vi "Multiple_Ramps_Trimming_Coil.vi"(0 "Trimming_Coil_Ramp_Error":dbl, 1 "Trimming_Coil_Ramp_Inc/Dec":dbl) -> ()   [LabVIEW 2025]
uses:
  Trimming_Coil_Command.vi
  Trimming_Coil_Ramps.vi
panel:
  out "TC1_Set_Point":dbl
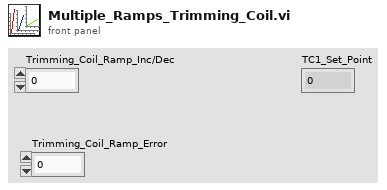
[diagram p1: front panel]
types:
  T1 = cluster{"TC1_Set_Point":dbl, "TC2_Set_Point":dbl, "TC3_Set_Point":dbl, "TC4_Set_Point":dbl, "TC5_Set_Point":dbl, "TC6_Set_Point":dbl, "TC7_Set_Point":dbl, "TC8_Set_Point":dbl, "TC9_Set_Point":dbl, "TC10_Set_Point":dbl, "TC11_Set_Point":dbl, "TC12_Set_Point":dbl}
  T2 = cluster{"TC1_Ramp":dbl, "TC2_Ramp":dbl, "TC3_Ramp":dbl, "TC4_Ramp":dbl, "TC5_Ramp":dbl, "TC6_Ramp":dbl, "TC7_Ramp":dbl, "TC8_Ramp":dbl, "TC9_Ramp":dbl, "TC10_Ramp":dbl, "TC11_Ramp":dbl, "TC12_Ramp":dbl}
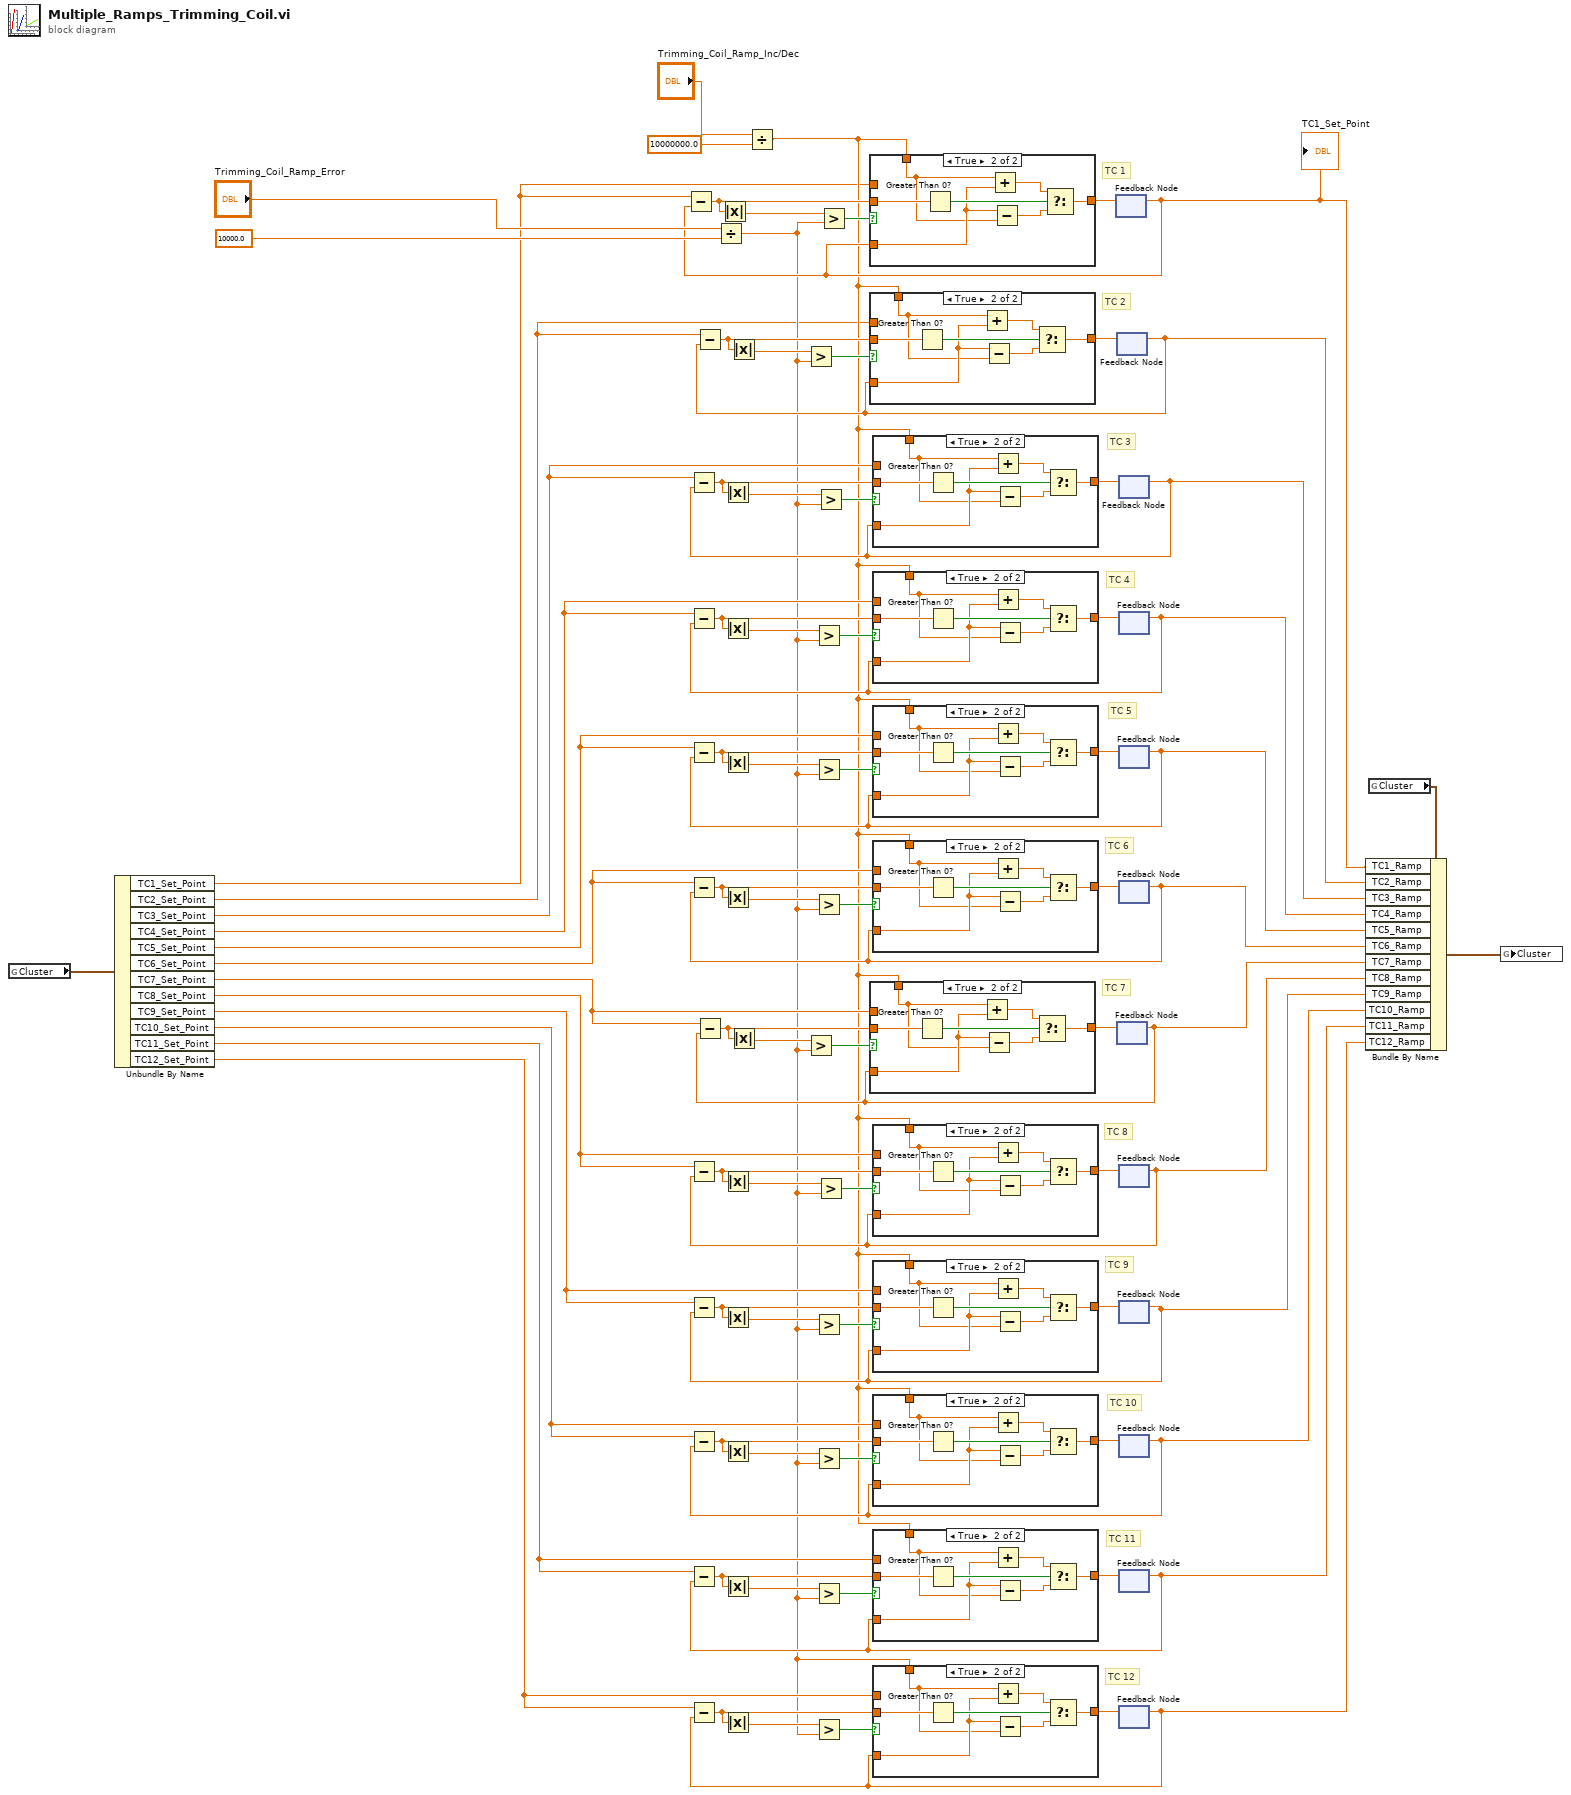
[diagram p0: block diagram]
diagram:
  # "TC 12"
  # "TC 11"
  # "TC 10"
  # "TC 9"
  # "TC 8"
  # "TC 7"
  # "TC 6"
  # "TC 5"
  # "TC 4"
  # "TC 3"
  # "TC 2"
  # "TC 1"
  n1 = global read "Trimming_Coil_Command.vi" "Cluster"() -> (w75:T1)
  n2 = Unbundle By Name(w75) -> ("TC1_Set_Point"=w1:dbl, "TC2_Set_Point"=w2:dbl, "TC3_Set_Point"=w63:dbl, "TC4_Set_Point"=w58:dbl, "TC5_Set_Point"=w49:dbl, "TC6_Set_Point"=w48:dbl, "TC7_Set_Point"=w24:dbl, "TC8_Set_Point"=w23:dbl, "TC9_Set_Point"=w22:dbl, "TC10_Set_Point"=w21:dbl, "TC11_Set_Point"=w20:dbl, "TC12_Set_Point"=w15:dbl)
  n3 = Divide(x="Trimming_Coil_Ramp_Error", y=10000.0) -> (x/y=w3:dbl)
  n4 = Divide(x="Trimming_Coil_Ramp_Inc/Dec", y=10000000.0) -> (x/y=w4:dbl)
  n5 = feedback #1() -> (w5:dbl)  [unwired: 1 in]
  "TC1_Set_Point" <- w5
  n6 = Subtract(x=w1, y=w5) -> (x-y=w80:dbl)
  n7 = Absolute Value(x=w80) -> (abs(x)=w81:dbl)
  n8 = Greater?(x=w81, y=w3) -> (0:w79:bool)
  n9 = case shown="True" w79 {
    tunnel: w80 -> [_ w89]
    tunnel: w5 -> [_ w87]
    tunnel: [w82 w84] -> w78
    tunnel: w1 -> [w82 _]
    tunnel: w4 -> [_ w83]
    frame False {
    }
    frame True {
      n10 = Greater Than 0?(x=w89) -> (x > 0?=w88:bool)
      n11 = Add(x=w83, y=w87) -> (x+y=w85:dbl)
      n12 = Subtract(x=w87, y=w83) -> (x-y=w86:dbl)
      n13 = Select(t=w85, s=w88, f=w86) -> (s? t:f=w84:dbl)
    }
  }
  n14 = feedback-in #1(w78) -> ()
  n15 = feedback #2() -> (w6:dbl)  [unwired: 1 in]
  n16 = Subtract(x=w2, y=w6) -> (x-y=w70:dbl)
  n17 = Absolute Value(x=w70) -> (abs(x)=w71:dbl)
  n18 = Greater?(x=w71, y=w3) -> (0:w69:bool)
  n19 = case shown="True" w69 {
    tunnel: w70 -> [_ w97]
    tunnel: w6 -> [_ w95]
    tunnel: [w90 w92] -> w68
    tunnel: w2 -> [w90 _]
    tunnel: w4 -> [_ w91]
    frame False {
    }
    frame True {
      n20 = Greater Than 0?(x=w97) -> (x > 0?=w96:bool)
      n21 = Add(x=w91, y=w95) -> (x+y=w93:dbl)
      n22 = Subtract(x=w95, y=w91) -> (x-y=w94:dbl)
      n23 = Select(t=w93, s=w96, f=w94) -> (s? t:f=w92:dbl)
    }
  }
  n24 = feedback-in #2(w68) -> ()
  n25 = feedback #3() -> (w14:dbl)  [unwired: 1 in]
  n26 = Subtract(x=w24, y=w14) -> (x-y=w43:dbl)
  n27 = Absolute Value(x=w43) -> (abs(x)=w44:dbl)
  n28 = Greater?(x=w44, y=w3) -> (0:w42:bool)
  n29 = case shown="True" w42 {
    tunnel: w43 -> [_ w105]
    tunnel: w14 -> [_ w103]
    tunnel: [w98 w100] -> w41
    tunnel: w24 -> [w98 _]
    tunnel: w4 -> [_ w99]
    frame False {
    }
    frame True {
      n30 = Greater Than 0?(x=w105) -> (x > 0?=w104:bool)
      n31 = Add(x=w99, y=w103) -> (x+y=w101:dbl)
      n32 = Subtract(x=w103, y=w99) -> (x-y=w102:dbl)
      n33 = Select(t=w101, s=w104, f=w102) -> (s? t:f=w100:dbl)
    }
  }
  n34 = feedback-in #3(w41) -> ()
  n35 = feedback #4() -> (w7:dbl)  [unwired: 1 in]
  n36 = Subtract(x=w63, y=w7) -> (x-y=w66:dbl)
  n37 = Absolute Value(x=w66) -> (abs(x)=w67:dbl)
  n38 = Greater?(x=w67, y=w3) -> (0:w65:bool)
  n39 = case shown="True" w65 {
    tunnel: w66 -> [_ w113]
    tunnel: w7 -> [_ w111]
    tunnel: [w106 w108] -> w64
    tunnel: w63 -> [w106 _]
    tunnel: w4 -> [_ w107]
    frame False {
    }
    frame True {
      n40 = Greater Than 0?(x=w113) -> (x > 0?=w112:bool)
      n41 = Add(x=w107, y=w111) -> (x+y=w109:dbl)
      n42 = Subtract(x=w111, y=w107) -> (x-y=w110:dbl)
      n43 = Select(t=w109, s=w112, f=w110) -> (s? t:f=w108:dbl)
    }
  }
  n44 = feedback-in #4(w64) -> ()
  n45 = feedback #5() -> (w47:dbl)  [unwired: 1 in]
  n46 = Subtract(x=w58, y=w47) -> (x-y=w61:dbl)
  n47 = Absolute Value(x=w61) -> (abs(x)=w62:dbl)
  n48 = Greater?(x=w62, y=w3) -> (0:w60:bool)
  n49 = case shown="True" w60 {
    tunnel: w61 -> [_ w121]
    tunnel: w47 -> [_ w119]
    tunnel: [w114 w116] -> w59
    tunnel: w58 -> [w114 _]
    tunnel: w4 -> [_ w115]
    frame False {
    }
    frame True {
      n50 = Greater Than 0?(x=w121) -> (x > 0?=w120:bool)
      n51 = Add(x=w115, y=w119) -> (x+y=w117:dbl)
      n52 = Subtract(x=w119, y=w115) -> (x-y=w118:dbl)
      n53 = Select(t=w117, s=w120, f=w118) -> (s? t:f=w116:dbl)
    }
  }
  n54 = feedback-in #5(w59) -> ()
  n55 = feedback #6() -> (w46:dbl)  [unwired: 1 in]
  n56 = Subtract(x=w49, y=w46) -> (x-y=w56:dbl)
  n57 = Absolute Value(x=w56) -> (abs(x)=w57:dbl)
  n58 = Greater?(x=w57, y=w3) -> (0:w55:bool)
  n59 = case shown="True" w55 {
    tunnel: w56 -> [_ w129]
    tunnel: w46 -> [_ w127]
    tunnel: [w122 w124] -> w54
    tunnel: w49 -> [w122 _]
    tunnel: w4 -> [_ w123]
    frame False {
    }
    frame True {
      n60 = Greater Than 0?(x=w129) -> (x > 0?=w128:bool)
      n61 = Add(x=w123, y=w127) -> (x+y=w125:dbl)
      n62 = Subtract(x=w127, y=w123) -> (x-y=w126:dbl)
      n63 = Select(t=w125, s=w128, f=w126) -> (s? t:f=w124:dbl)
    }
  }
  n64 = feedback-in #6(w54) -> ()
  n65 = feedback #7() -> (w45:dbl)  [unwired: 1 in]
  n66 = Subtract(x=w48, y=w45) -> (x-y=w52:dbl)
  n67 = Absolute Value(x=w52) -> (abs(x)=w53:dbl)
  n68 = Greater?(x=w53, y=w3) -> (0:w51:bool)
  n69 = case shown="True" w51 {
    tunnel: w52 -> [_ w137]
    tunnel: w45 -> [_ w135]
    tunnel: [w130 w132] -> w50
    tunnel: w48 -> [w130 _]
    tunnel: w4 -> [_ w131]
    frame False {
    }
    frame True {
      n70 = Greater Than 0?(x=w137) -> (x > 0?=w136:bool)
      n71 = Add(x=w131, y=w135) -> (x+y=w133:dbl)
      n72 = Subtract(x=w135, y=w131) -> (x-y=w134:dbl)
      n73 = Select(t=w133, s=w136, f=w134) -> (s? t:f=w132:dbl)
    }
  }
  n74 = feedback-in #7(w50) -> ()
  n75 = feedback #8() -> (w13:dbl)  [unwired: 1 in]
  n76 = Subtract(x=w23, y=w13) -> (x-y=w39:dbl)
  n77 = Absolute Value(x=w39) -> (abs(x)=w40:dbl)
  n78 = Greater?(x=w40, y=w3) -> (0:w38:bool)
  n79 = case shown="True" w38 {
    tunnel: w39 -> [_ w145]
    tunnel: w13 -> [_ w143]
    tunnel: [w138 w140] -> w37
    tunnel: w23 -> [w138 _]
    tunnel: w4 -> [_ w139]
    frame False {
    }
    frame True {
      n80 = Greater Than 0?(x=w145) -> (x > 0?=w144:bool)
      n81 = Add(x=w139, y=w143) -> (x+y=w141:dbl)
      n82 = Subtract(x=w143, y=w139) -> (x-y=w142:dbl)
      n83 = Select(t=w141, s=w144, f=w142) -> (s? t:f=w140:dbl)
    }
  }
  n84 = feedback-in #8(w37) -> ()
  n85 = feedback #9() -> (w12:dbl)  [unwired: 1 in]
  n86 = Subtract(x=w22, y=w12) -> (x-y=w35:dbl)
  n87 = Absolute Value(x=w35) -> (abs(x)=w36:dbl)
  n88 = Greater?(x=w36, y=w3) -> (0:w34:bool)
  n89 = case shown="True" w34 {
    tunnel: w35 -> [_ w153]
    tunnel: w12 -> [_ w151]
    tunnel: [w146 w148] -> w33
    tunnel: w22 -> [w146 _]
    tunnel: w4 -> [_ w147]
    frame False {
    }
    frame True {
      n90 = Greater Than 0?(x=w153) -> (x > 0?=w152:bool)
      n91 = Add(x=w147, y=w151) -> (x+y=w149:dbl)
      n92 = Subtract(x=w151, y=w147) -> (x-y=w150:dbl)
      n93 = Select(t=w149, s=w152, f=w150) -> (s? t:f=w148:dbl)
    }
  }
  n94 = feedback-in #9(w33) -> ()
  n95 = feedback #10() -> (w11:dbl)  [unwired: 1 in]
  n96 = Subtract(x=w21, y=w11) -> (x-y=w31:dbl)
  n97 = Absolute Value(x=w31) -> (abs(x)=w32:dbl)
  n98 = Greater?(x=w32, y=w3) -> (0:w30:bool)
  n99 = case shown="True" w30 {
    tunnel: w31 -> [_ w161]
    tunnel: w11 -> [_ w159]
    tunnel: [w154 w156] -> w29
    tunnel: w21 -> [w154 _]
    tunnel: w4 -> [_ w155]
    frame False {
    }
    frame True {
      n100 = Greater Than 0?(x=w161) -> (x > 0?=w160:bool)
      n101 = Add(x=w155, y=w159) -> (x+y=w157:dbl)
      n102 = Subtract(x=w159, y=w155) -> (x-y=w158:dbl)
      n103 = Select(t=w157, s=w160, f=w158) -> (s? t:f=w156:dbl)
    }
  }
  n104 = feedback-in #10(w29) -> ()
  n105 = feedback #11() -> (w10:dbl)  [unwired: 1 in]
  n106 = Subtract(x=w20, y=w10) -> (x-y=w27:dbl)
  n107 = Absolute Value(x=w27) -> (abs(x)=w28:dbl)
  n108 = Greater?(x=w28, y=w3) -> (0:w26:bool)
  n109 = case shown="True" w26 {
    tunnel: w27 -> [_ w169]
    tunnel: w10 -> [_ w167]
    tunnel: [w162 w164] -> w25
    tunnel: w20 -> [w162 _]
    tunnel: w4 -> [_ w163]
    frame False {
    }
    frame True {
      n110 = Greater Than 0?(x=w169) -> (x > 0?=w168:bool)
      n111 = Add(x=w163, y=w167) -> (x+y=w165:dbl)
      n112 = Subtract(x=w167, y=w163) -> (x-y=w166:dbl)
      n113 = Select(t=w165, s=w168, f=w166) -> (s? t:f=w164:dbl)
    }
  }
  n114 = feedback-in #11(w25) -> ()
  n115 = feedback #12() -> (w9:dbl)  [unwired: 1 in]
  n116 = Subtract(x=w15, y=w9) -> (x-y=w18:dbl)
  n117 = Absolute Value(x=w18) -> (abs(x)=w19:dbl)
  n118 = Greater?(x=w19, y=w3) -> (0:w17:bool)
  n119 = case shown="True" w17 {
    tunnel: w18 -> [_ w177]
    tunnel: w9 -> [_ w175]
    tunnel: [w170 w172] -> w16
    tunnel: w15 -> [w170 _]
    tunnel: w3 -> [_ w171]
    frame False {
    }
    frame True {
      n120 = Greater Than 0?(x=w177) -> (x > 0?=w176:bool)
      n121 = Add(x=w171, y=w175) -> (x+y=w173:dbl)
      n122 = Subtract(x=w175, y=w171) -> (x-y=w174:dbl)
      n123 = Select(t=w173, s=w176, f=w174) -> (s? t:f=w172:dbl)
    }
  }
  n124 = feedback-in #12(w16) -> ()
  n125 = global read "Trimming_Coil_Ramps.vi" "Cluster"() -> (w74:T2)
  n126 = Bundle By Name(cluster=w74, "TC1_Ramp"=w5, "TC2_Ramp"=w6, "TC3_Ramp"=w7, "TC4_Ramp"=w47, "TC5_Ramp"=w46, "TC6_Ramp"=w45, "TC7_Ramp"=w14, "TC8_Ramp"=w13, "TC9_Ramp"=w12, "TC10_Ramp"=w11, "TC11_Ramp"=w10, "TC12_Ramp"=w9) -> (w8:T2)
  n127 = global write "Trimming_Coil_Ramps.vi" "Cluster"(w8) -> ()
